vi "TblAddParam (SubVI).vi"(8 "error in":errorcluster) -> (0 "error out":errorcluster, 2 "Tbl1Param":sgl[][](array[numeric]), 3 "Tbl0Param":sgl[][](array[numeric]))   [LabVIEW 2017]
uses:
  Global_SNK3_HF.vi
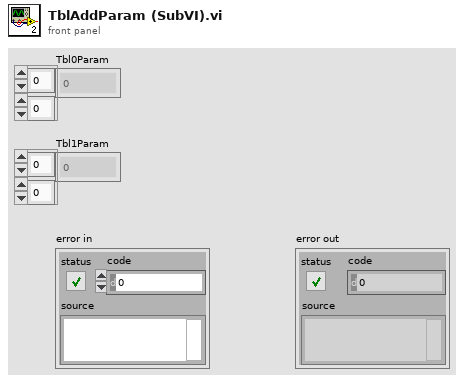
[diagram p1: front panel]
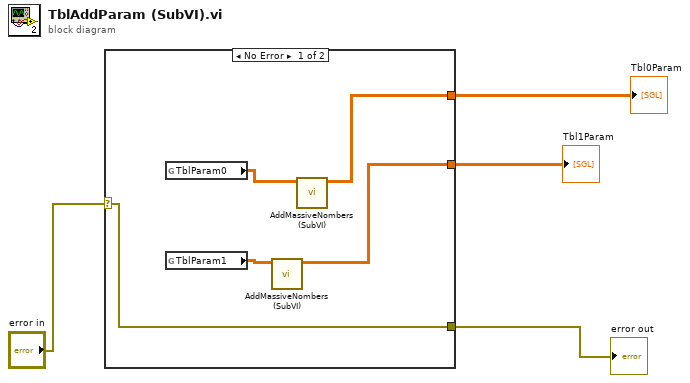
[diagram p0: block diagram]
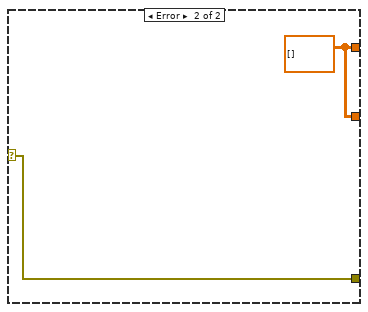
[diagram p2: hidden frame]
diagram:
  n1 = case shown="No Error" "error in" {
    selector: "error in" -> [w5 w10]
    tunnel: [w9 w11] -> w4
    tunnel: [w7 w11] -> w3
    tunnel: [w5 w10] -> w1
    frame No Error {
      n2 = global read "Global_SNK3_HF.vi" "TblParam0"() -> (w6:sgl[][])
      n3 = global read "Global_SNK3_HF.vi" "TblParam1"() -> (w8:sgl[][])
      n4 = call "AddMassiveNombers (SubVI).vi"("TblParam in"=w8) -> ("TblParam out"=w9:sgl[][])  [unwired: 10 in]
      n5 = call "AddMassiveNombers (SubVI).vi"("TblParam in"=w6) -> ("TblParam out"=w7:sgl[][])  [unwired: 10 in]
    }
    frame Error {
      w11 = sgl[][] [] ("TblParam out")
    }
  }
  "Tbl1Param" <- w4
  "Tbl0Param" <- w3
  "error out" <- w1
